vi "SaveChannels.vi"(8 "error in (no error)":errorcluster, 11 "object in":refnum<class "ChannelsManager.lvclass">) -> (0 "error out":errorcluster, 3 "object out":refnum<class "ChannelsManager.lvclass">)   [LabVIEW 2021, in "Channel.lvlib" / "ChannelsManager.lvlib" / "ChannelsManager.lvclass"]
uses:
  ChannelsManager.lvclass
  ChannelsManager.lvclass/ChannelsManager.ctl
  Channel_class/Channel.lvclass
  Channel.lvlib
  <vilib>/Utility/config.llb/NI_LVConfig.lvlib
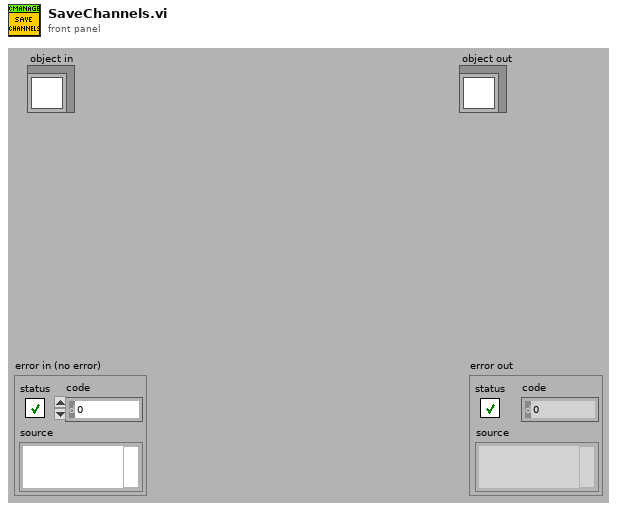
[diagram p1: front panel]
types:
  T1 = typedef "NI_LVConfig.lvlib/Config Data RefNum.ctl" = refnum<k1>
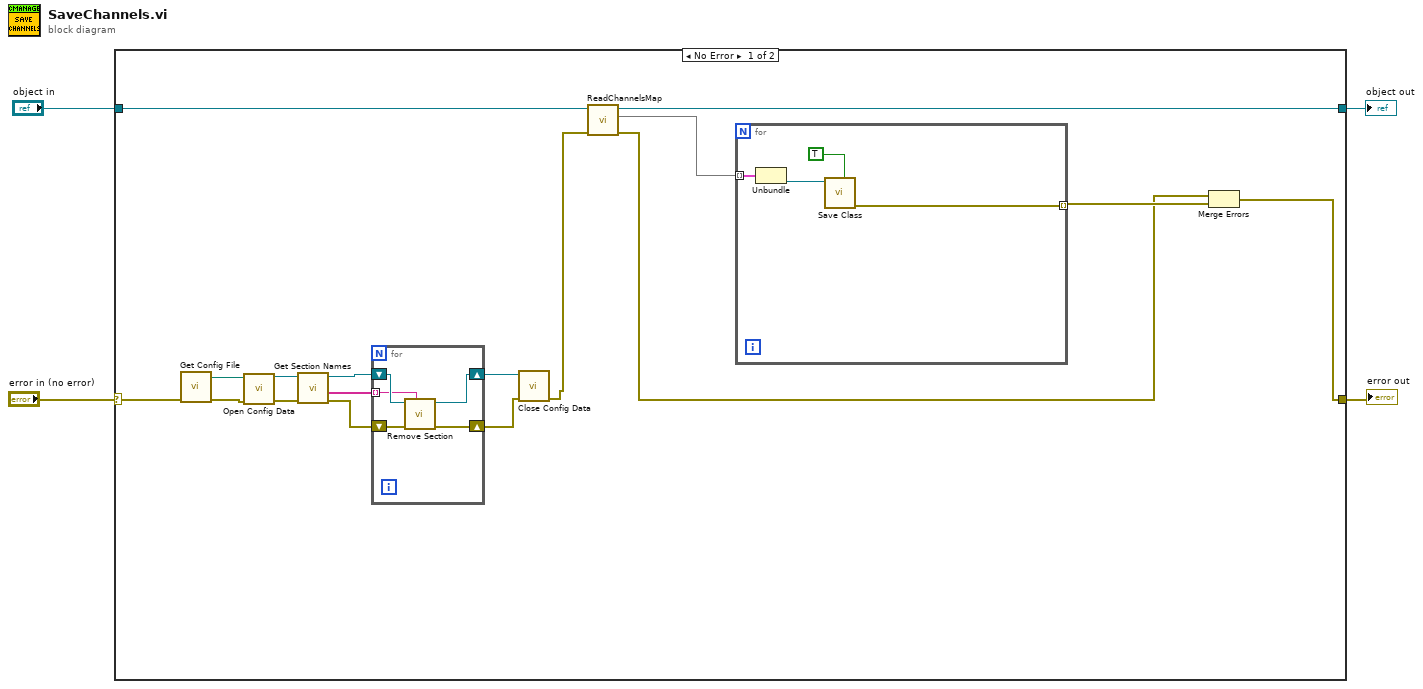
[diagram p0: block diagram]
diagram:
  n1 = case shown="No Error" "error in (no error)" {
    selector: "error in (no error)" -> [w15 w32]
    tunnel: [w16 w32] -> w3
    tunnel: [w20 w31] -> w1
    tunnel: "object in" -> [w21 w31]
    frame No Error {
      n2 = call "Get Config File.vi"("error in (no error)"=w15) -> ("error out"=w12:errorcluster, "Config File"=w11:path)  [unwired: 9 in]
      n3 = call <vilib>:"Open Config Data.vi"("error in (no error)"=w12, "configuration file path"=w11) -> ("error out"=w14:errorcluster, "refnum"=w13:T1)  [unwired: 7 in, 1 out]
      n4 = call <vilib>:"Get Section Names.vi"("error in (no error)"=w14, "refnum"=w13) -> ("error out"=w7:errorcluster, "section names"=w5:string[], "refnum out"=w10:T1)  [unwired: 7 in]
      n5 = for {
        shift-right: [w23] -> w6
        shift-left: w10 -> [w26]
        shift-right: [w25] -> w8
        shift-left: w7 -> [w24]
        tunnel: w5 -> [w22] mode=indexing
        n6 = call <vilib>:"Remove Section.vi"("section"=w22, "error in (no error)"=w24, "refnum"=w26) -> ("error out"=w25:errorcluster, "refnum out"=w23:T1)  [unwired: 6 in, 1 out]
      }
      n7 = call <vilib>:"Close Config Data.vi"("error in (no error)"=w8, "refnum"=w6) -> ("error out"=w9:errorcluster)  [unwired: 8 in, 1 out]
      n8 = call-dynamic "ReadChannelsMap.vi"("error in (no error)"=w9, "object in"=w21) -> ("error out"=w17:errorcluster, "Channels Map"=w19:map{string, refnum<class "Channel.lvclass">}, "object out"=w20:refnum<class "ChannelsManager.lvclass">)  [unwired: 7 in]
      n9 = for {
        tunnel: w19 -> [w30] mode=indexing
        tunnel: [w27] -> w18 mode=indexing
        n10 = Unbundle(w30) -> ("Channel"=w29:refnum<class "Channel.lvclass">)  [unwired: 1 out]
        n11 = call "Save Class.vi"("Clear Before Saving(F)"=TRUE, "Channel"=w29) -> ("error out"=w27:errorcluster)  [unwired: 8 in, 1 out]
      }
      n12 = Merge Errors(w17, w18) -> (w16:errorcluster)
    }
    frame Error {
    }
  }
  "error out" <- w3
  "object out" <- w1
